vi "ToolBarButtonDraw.vi"(8 "error in (no error)":errorcluster, 9 "Coords":T1, 11 "Gviewer in":refnum<class "Gviewer.lvclass">) -> (0 "error out":errorcluster, 3 "Gviewer out":refnum<class "Gviewer.lvclass">)   [LabVIEW 2020, in "Sgraph_lib_V1.lvlib" / "Gviewer.lvclass"]
doc: "Draw toolbar buttons and objects on mouse move"
uses:
  Gviewer.lvclass
  <vilib>/Utility/miscctls.llb/LVPoint32TypeDef.ctl
  Gviewer.lvclass/Gviewer.ctl
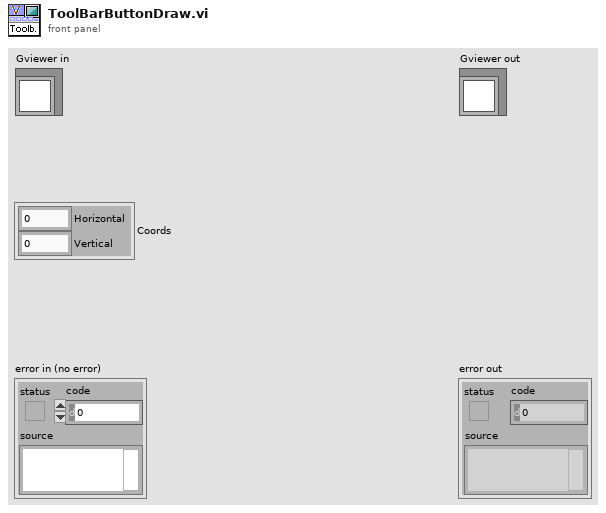
[diagram p1: front panel]
types:
  T1 = typedef "LVPoint32TypeDef.ctl" = cluster{"Horizontal":i32, "Vertical":i32}
  T2 = cluster{"left":i16, "top":i16, "right":i16, "bottom":i16}
  T3 = cluster{"horizontal":enum16{"left", "center", "right"}, "vertical":enum16{"top", "center", "bottom"}}
  T4 = typedef "Sgraph_lib_V1.lvlib/Gviewer.lvclass/Typedef_ZoomEvent.ctl" = cluster{"Time-Start":timestamp, "Time-End":timestamp, "TimeSpan(sec)":dbl, "Live":T5, "SelProperties":T6[], "Time Stamp":timestamp}
  T5 = typedef "Sgraph_lib_V1.lvlib/Gviewer.lvclass/Typedef_Live.ctl" = enum16{"Live View", "Freeze"}
  T6 = typedef "Sgraph_lib_V1.lvlib/Gviewer.lvclass/Typedef_SelProperties.ctl" = cluster{"Color":u32, "LineType":T7, "max":dbl, "min":dbl}
  T7 = typedef "Sgraph_lib_V1.lvlib/Gviewer.lvclass/Typedef_LineType.ctl" = enum16{"num_bare", "num_MinMax_Area", "num_MinMax_Lines", "num_MinMax_Forfor", "num_Max_Area", "num_Max_Line", "num_Max_Forfor", "num_Min_Area", "num_Min_Line", "num_Min_Fosfor", "Boolean_Line_01", "Boolean_Area_01", "Boolean_Fosfor_01", "Boolean_Line_TF", "Boolean_Area_TF", "Boolean_Fosfor_TF", "Boolean_OnOff_Line", "Boolean_OnOff_Area", "Boolean_OnOff_Fosfor", "Boolean_spare", "StringEvent_Line", "StringEvent_TimeLine"}
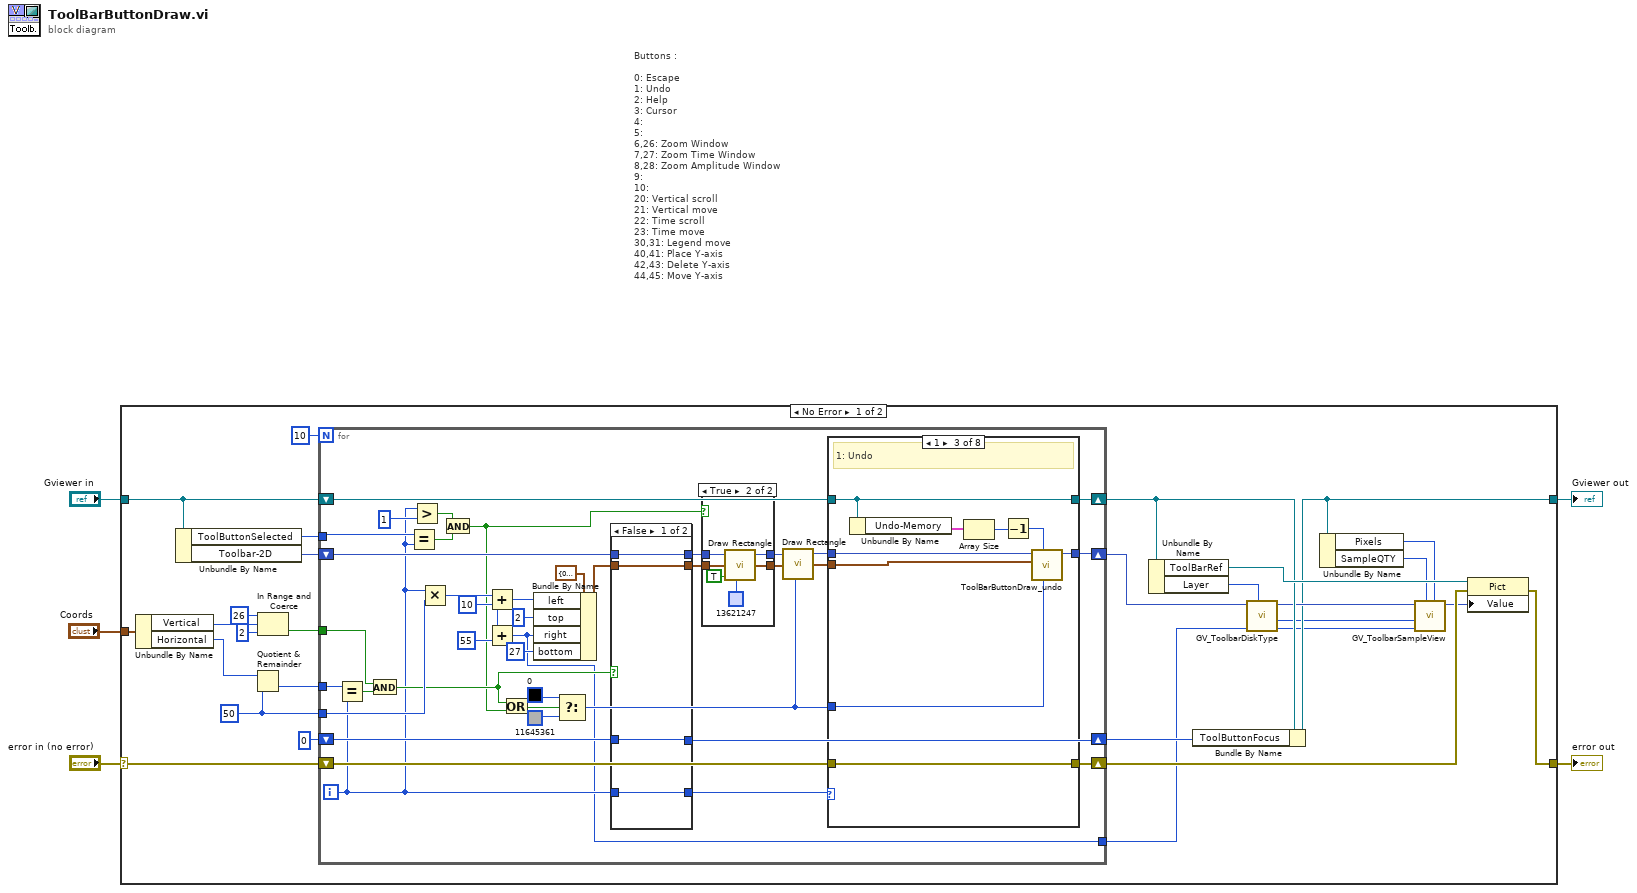
[diagram p0: block diagram]
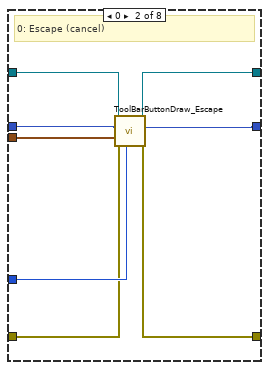
[diagram p3: hidden frame]
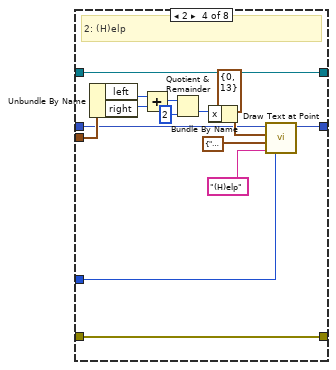
[diagram p4: hidden frame]
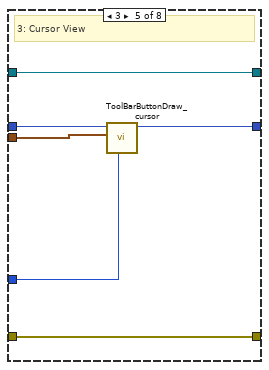
[diagram p5: hidden frame]
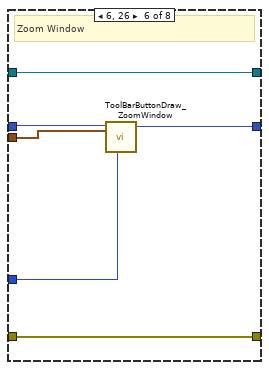
[diagram p6: hidden frame]
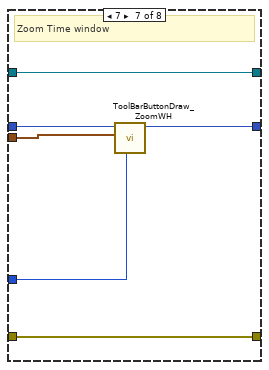
[diagram p7: hidden frame]
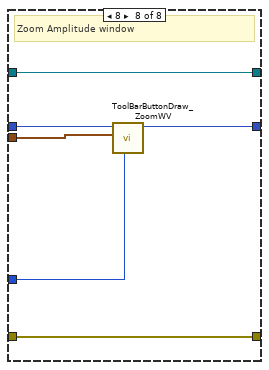
[diagram p8: hidden frame]
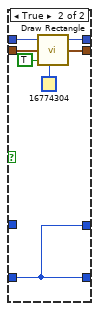
[diagram p10: hidden frame]
diagram:
  # "Buttons :\n\n0: Escape\n1: Undo\n2: Help\n3: Cursor\n4: \n5:\n6,26: Zoom Window\n7,27: Zoom Time Window\n8,28: Zoom Amplitude Window\n9:\n10:\n20: Vertical scroll\n21: Vertical move\n22: Time scroll\n23: Time move\n30,31: Legend move\n40,41: Place Y-axis\n42,43: Delete Y-axis\n44,45: Move Y-axis"
  n1 = case shown="No Error" "error in (no error)" {
    selector: "error in (no error)" -> [w34 w150]
    tunnel: [w28 w150] -> w4
    tunnel: [w10 w149] -> w2
    tunnel: "Gviewer in" -> [w33 w149]
    tunnel: "Coords" -> [w27 _]
    frame No Error {
      w21 = 50 ("y")
      n2 = Unbundle By Name(w27) -> ("Vertical"=w26:i32, "Horizontal"=w22:i32)
      n3 = Unbundle By Name(w33) -> ("ToolButtonSelected"=w19:i32, "Toolbar-2D"=w32:picture)
      n4 = Quotient & Remainder(x=w22, y=w21) -> (floor(x/y)=w20:i32)  [unwired: 1 out]
      n5 = In Range and Coerce(upper limit=26, x=w26, lower limit=2) -> (In Range?=w23:bool)  [unwired: 1 out]
      n6 = for {
        N: 10 -> [_]
        shift-right: [w46] -> w16
        shift-left: w33 -> [w47]
        shift-right: [w42] -> w29
        shift-left: w34 -> [w43]
        shift-right: [w44] -> w15
        shift-left: w32 -> [w59]
        tunnel: w23 -> [w62]
        tunnel: w21 -> [w65]
        tunnel: w20 -> [w64]
        tunnel: w19 -> [w54]
        shift-right: [w39] -> w17
        shift-left: 0 -> [w40]
        tunnel: [w35] -> w11
        i -> [w38]
        n7 = Equal?(x=w64, y=w38) -> (x = y?=w63:bool)
        n8 = And(x=w62, y=w63) -> (x .and. y?=w49:bool)
        n9 = Equal?(x=w54, y=w38) -> (x = y?=w52:bool)
        n10 = Greater?(x=w38, y=1 ("x")) -> (0:w53:bool)
        n11 = Multiply(x=w38, y=w65) -> (x*y=w69:i32)
        n12 = And(x=w53, y=w52) -> (x .and. y?=w48:bool)
        n13 = Add(x=w69, y=10) -> (x+y=w66:i32)
        n14 = Add(x=w69, y=55) -> (x+y=w35:i32)
        n15 = Or(x=w49, y=w48) -> (x .or. y?=w50:bool)
        n16 = Bundle By Name(cluster=T2 {"left"=0, "top"=0, "right"=0, "bottom"=0} ("rect"), "left"=w66, "top"=i16 2, "right"=w35, "bottom"=i16 27) -> (w58:T2)
        n17 = Select(t=u32 0, s=w50, f=u32 11645361) -> (s? t:f=w41:u32)
        n18 = case shown="False" w49 {
          tunnel: w59 -> [w142 w148]
          tunnel: [w142 w147] -> w57
          tunnel: w58 -> [w141 w146]
          tunnel: [w141 w146] -> w55
          tunnel: w40 -> [w140 _]
          tunnel: [w140 w143] -> w39
          tunnel: w38 -> [w139 w143]
          tunnel: [w139 w143] -> w37
          frame False {
          }
          frame True {
            n19 = call <vilib>:"Draw Rectangle.vi"("picture"=w148, "rect"=w146, "fill?(F)"=TRUE, "color(black)"=u32 16774304) -> ("new picture"=w147:picture)  [unwired: 5 in]
          }
        }
        n20 = case shown="True" w48 {
          tunnel: w57 -> [w133 w137]
          tunnel: [w133 w136] -> w56
          tunnel: w55 -> [w132 w138]
          tunnel: [w132 w138] -> w36
          frame False {
          }
          frame True {
            n21 = call <vilib>:"Draw Rectangle.vi"("picture"=w137, "rect"=w138, "fill?(F)"=TRUE, "color(black)"=u32 13621247) -> ("new picture"=w136:picture)  [unwired: 5 in]
          }
        }
        n22 = call <vilib>:"Draw Rectangle.vi"("picture"=w56, "rect"=w36, "color(black)"=w41) -> ("new picture"=w45:picture)  [unwired: 6 in]
        n23 = case shown="1" w37 {
          tunnel: w47 -> [w75 w80 w87 w107 w113 w119 w125 w131]
          tunnel: [w75 w81 w87 w107 w113 w119 w125 w131] -> w46
          tunnel: w45 -> [w74 w77 w91 w93 w112 w117 w123 w129]
          tunnel: [w74 w76 w90 w105 w108 w116 w122 w128] -> w44
          tunnel: w43 -> [w73 w78 w92 w106 w109 w118 w124 w130]
          tunnel: [w73 w79 w92 w106 w109 w118 w124 w130] -> w42
          tunnel: w41 -> [_ w82 w88 w104 w110 w114 w120 w126]
          tunnel: w36 -> [_ w83 w89 w99 w111 w115 w121 w127]
          frame Default {
            # "Not implemented"
          }
          frame 0 {
            # "0: Escape (cancel)"
            n24 = call "ToolBarButtonDraw_Escape.vi"("Color"=w82, "error in"=w78, "rect"=w83, "Pict IN"=w77, "Gviewer in"=w80) -> ("error out"=w79:errorcluster, "Pict OUT"=w76:picture, "Gviewer out"=w81:refnum<class "Gviewer.lvclass">)  [unwired: 4 in]
          }
          frame 1 {
            # "1: Undo"
            n25 = Unbundle By Name(w87) -> ("Undo-Memory"=w86:T4[])
            n26 = Array Size(array=w86) -> (size(s)=w85:i32)
            n27 = Decrement(x=w85) -> (x-1=w84:i32)
            n28 = call "ToolBarButtonDraw_undo.vi"("Color"=w88, "undo size"=w84, "rect"=w89, "Pict IN"=w91) -> ("Pict OUT"=w90:picture)  [unwired: 7 in]
          }
          frame 2 {
            # "2: (H)elp"
            n29 = Unbundle By Name(w99) -> ("left"=w98:i16, "right"=w97:i16)
            n30 = Add(x=w98, y=w97) -> (x+y=w96:i16)
            n31 = Quotient & Remainder(x=w96, y=i16 2) -> (floor(x/y)=w94:i16)  [unwired: 1 out]
            n32 = Bundle By Name(cluster=cluster{"x":i16, "y":i16} {"x"=0, "y"=13} ("origin"), "x"=w94) -> (w101:cluster{"x":i16, "y":i16})
            n33 = call <vilib>:"Draw Text at Point.vi"("text color(black)"=w104, "text"="(H)elp", "alignment(left, top)"=T3 {"horizontal"=enum."center", "vertical"=enum."center"}, "origin"=w101, "picture"=w93) -> ("new picture"=w105:picture)  [unwired: 5 in, 1 out]
          }
          frame 3 {
            # "3: Cursor View"
            n34 = call "ToolBarButtonDraw_cursor.vi"("Color"=w110, "rect"=w111, "Pict IN"=w112) -> ("Pict OUT"=w108:picture)  [unwired: 8 in]
          }
          frame 6, 26 {
            # "Zoom Window"
            n35 = call "ToolBarButtonDraw_ZoomWindow.vi"("Color"=w114, "rect"=w115, "Pict IN"=w117) -> ("Pict OUT"=w116:picture)  [unwired: 8 in]
          }
          frame 7 {
            # "Zoom Time window"
            n36 = call "ToolBarButtonDraw_ZoomWH.vi"("Color"=w120, "rect"=w121, "Pict IN"=w123) -> ("Pict OUT"=w122:picture)  [unwired: 8 in]
          }
          frame 8 {
            # "Zoom Amplitude window"
            n37 = call "ToolBarButtonDraw_ZoomWV.vi"("Color"=w126, "rect"=w127, "Pict IN"=w129) -> ("Pict OUT"=w128:picture)  [unwired: 8 in]
          }
        }
      }
      n38 = Unbundle By Name(w16) -> ("ToolBarRef"=w30:refnum<vi>, "Layer"=w14:i32)
      n39 = Bundle By Name(cluster=w16, "ToolButtonFocus"=w17) -> (w10:refnum<class "Gviewer.lvclass">)
      n40 = call "GV_ToolbarDiskType.vi"("Layer"=w14, "Hor-pos"=w11, "Pict in"=w15) -> ("x"=w7:i16, "y"=w8:i16, "Pict out"=w13:picture)  [unwired: 6 in]
      n41 = Unbundle By Name(w10) -> ("Pixels"=w6:i32, "SampleQTY"=w9:i32)
      n42 = call "GV_ToolbarSampleView.vi"("Pixels"=w6, "Samples"=w9, "Hor-pos"=w7, "y"=w8, "Pict in"=w13) -> ("Pict out"=w12:picture)  [unwired: 6 in]
      n43 = property class="Pict"(reference=w30, error in=w29, "Value"=w12) -> (error out=w28:errorcluster)  [unwired: 1 out]
    }
    frame Error {
    }
  }
  "error out" <- w4
  "Gviewer out" <- w2
